vi "thermalCamera.vi"() -> ()   [LabVIEW 2025]
panel:
  out "Image":T1(plugin-control)
  out "IP address":string
  out "Output":string
  in  "Flag":bool
  in  "Stop recording":bool
  in  "Stop Preview":bool
  in  "Focus":dbl(slide) scale=0.0..100.0
  in  "Record":bool
  out "?":string
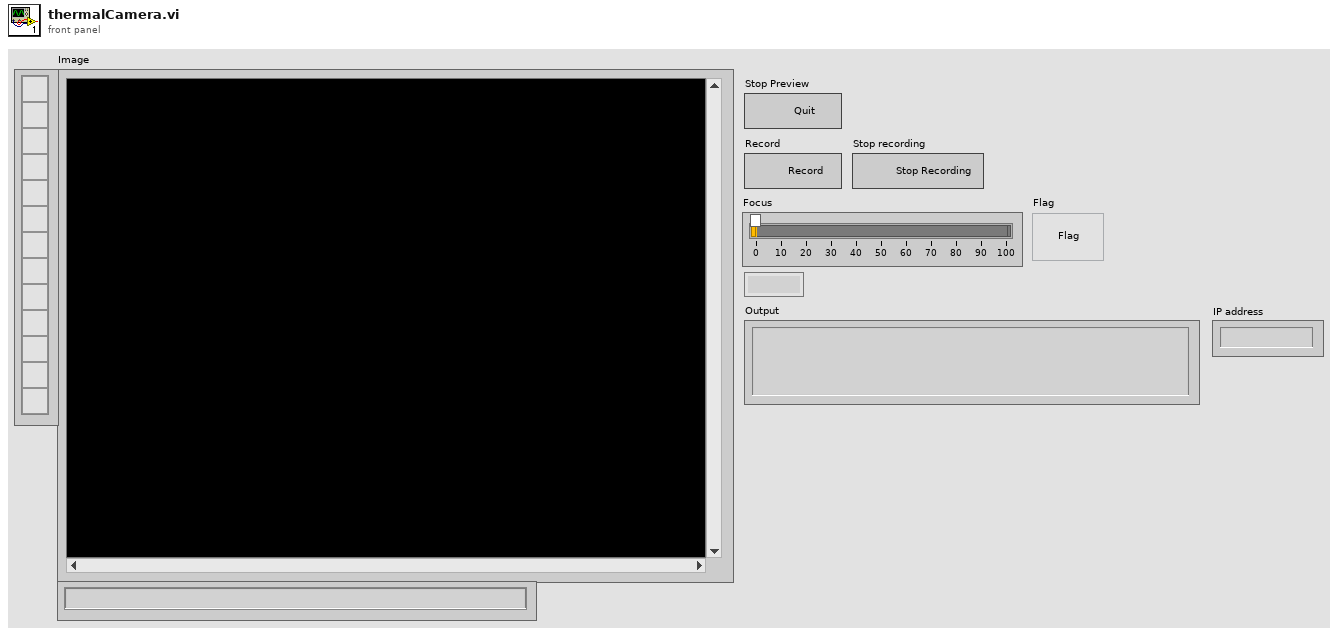
[diagram p1: front panel]
types:
  T1 = typedef "IMAQ Image.ctl" = refnum<image>
  T2 = enum16{"open", "replace", "create", "open or create", "replace or create", "replace or create with confirmation"}
  T3 = enum16{"big-endian, network order", "native, host order", "little-endian"}
  T4 = enum16{"Standard", "Buffered", "CRLF", "Immediate"}
  T5 = typedef "Image Type" = u32
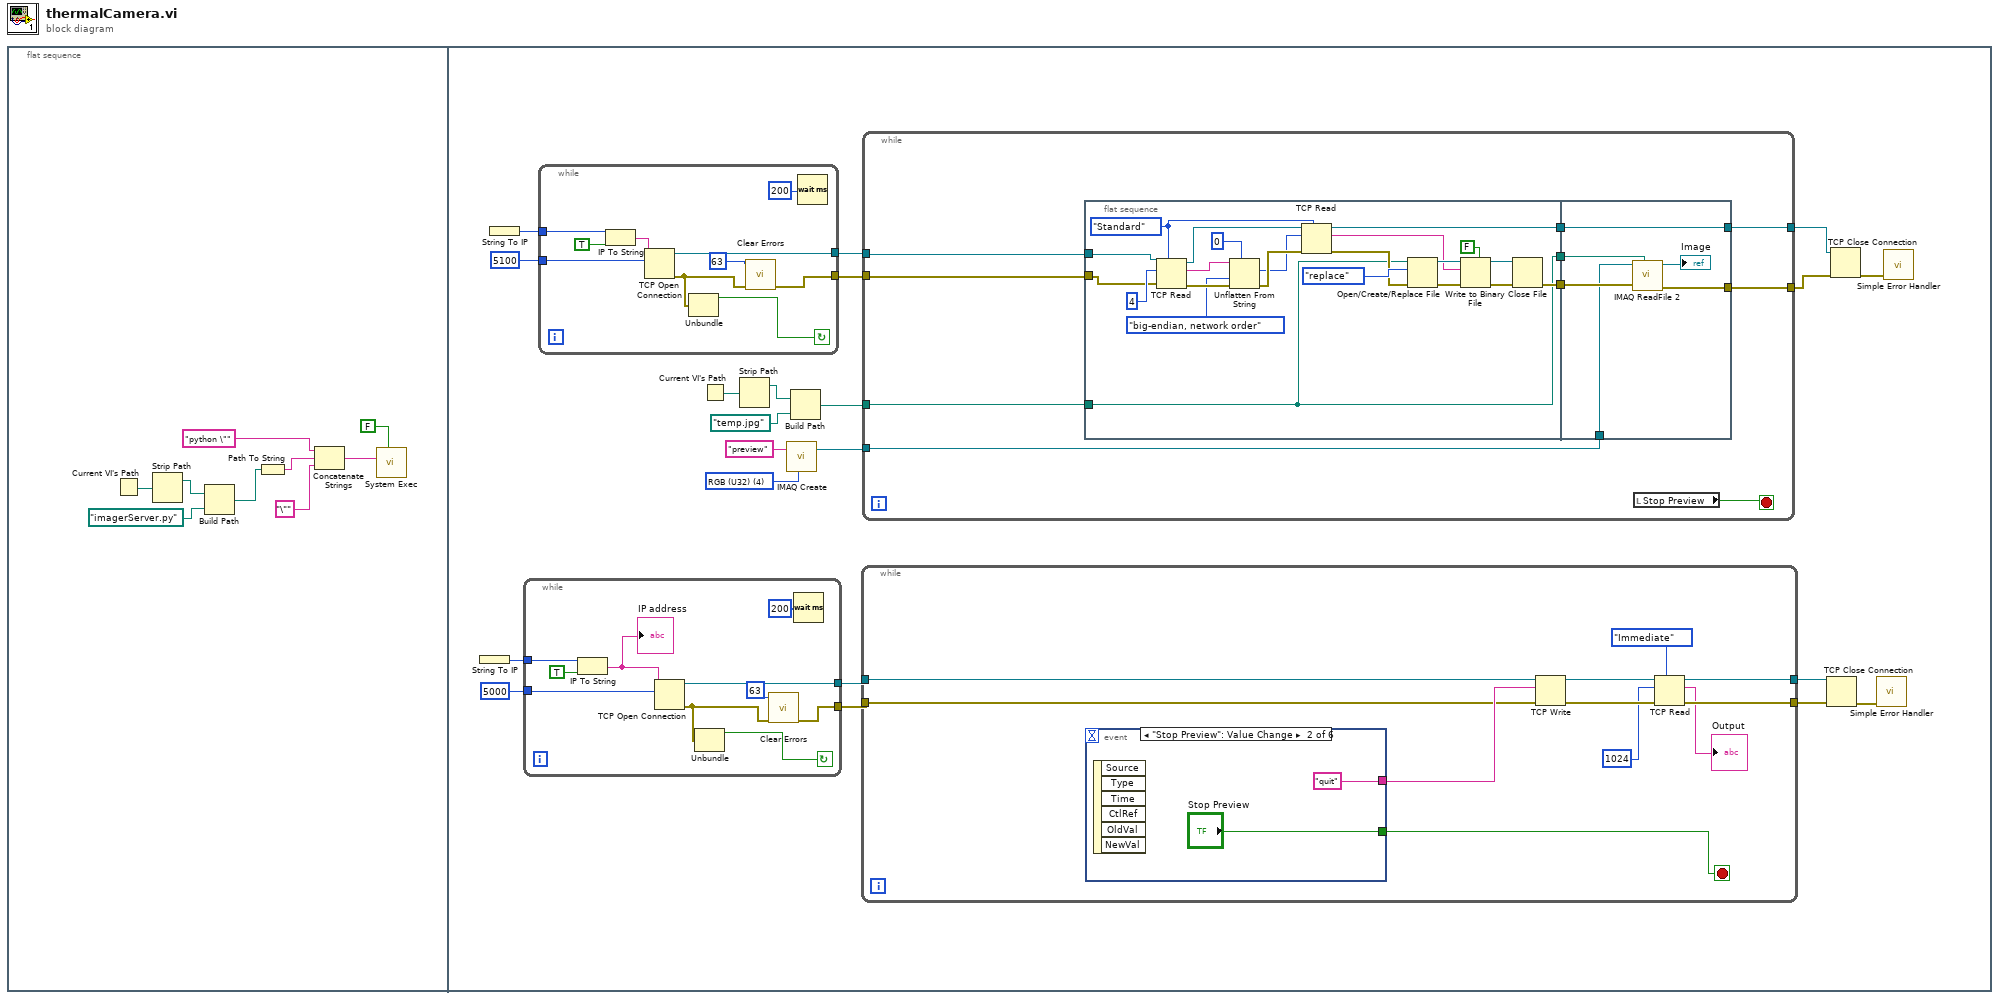
[diagram p0: block diagram]
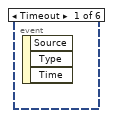
[diagram p2: hidden frame]
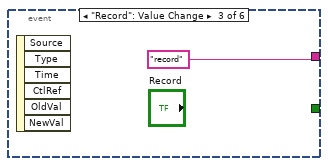
[diagram p3: hidden frame]
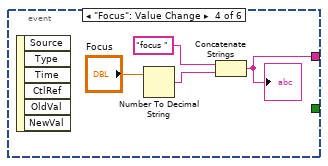
[diagram p4: hidden frame]
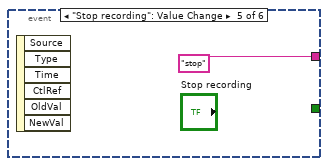
[diagram p5: hidden frame]
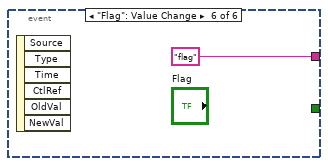
[diagram p6: hidden frame]
diagram:
  n1 = flat-sequence {
    frame #0 {
      n2 = Current VI's Path() -> (path=w4:path)
      n3 = Strip Path(path=w4) -> (stripped path=w5:path)  [unwired: 1 out]
      n4 = Build Path(base path=w5, name or relative path=path "imagerServer.py") -> (appended path=w2:path)
      n5 = Path To String(path=w2) -> (string=w8:string)
      n6 = Concatenate Strings("python \"" ("string"), w8, "\"" ("string")) -> (w7:string)
      n7 = call <vilib>:"System Exec.vi"("wait until completion? (T)"=FALSE, "command line"=w7) -> ()  [unwired: 6 in, 4 out]
    }
    frame #1 {
      w18 = T5 4 items=["Grayscale (U8)", "Grayscale (I16)", "Grayscale (SGL)", "Complex (CSG)", "RGB (U32)", "HSL (U32)", "RGB (U64)", "Grayscale (U16)"] ("Image Type")
      n8 = String To IP() -> (0:w15:u32)  [unwired: 1 in]
      n9 = String To IP() -> (0:w13:u32)  [unwired: 1 in]
      n10 = while {
        tunnel: [w44] -> w17
        tunnel: [w50] -> w16
        tunnel: w15 -> [w48]
        tunnel: u16 5000 ("remote port or service name") -> [w46]
        stop <- w41 continue-if-true
        n11 = IP To String(1:TRUE ("dot notation? (F)"), 2:w48) -> (0:w49:string)
        "IP address" <- w49
        n12 = TCP Open Connection(address=w49, remote port or service name=w46) -> (connection ID=w50:refnum<k5>, error out=w45:errorcluster)  [unwired: 3 in]
        n13 = Unbundle(w45) -> ("status"=w41:bool)  [unwired: 2 out]
        n14 = call <vilib>:"Clear Errors.vi"("error in (no error)"=w45, "specific error code to clear (0: all)"=63) -> ("error out"=w44:errorcluster)  [unwired: 4 in, 1 out]
        n15 = Wait (ms)(milliseconds to wait=u32 200) -> ()  [unwired: 1 out]
      }
      n16 = while {
        tunnel: w13 -> [w40]
        tunnel: [w34] -> w12
        tunnel: [w38] -> w11
        tunnel: u16 5100 ("remote port or service name") -> [w36]
        stop <- w31 continue-if-true
        n17 = IP To String(1:TRUE ("dot notation? (F)"), 2:w40) -> (0:w39:string)
        n18 = TCP Open Connection(address=w39, remote port or service name=w36) -> (connection ID=w38:refnum<k5>, error out=w35:errorcluster)  [unwired: 3 in]
        n19 = Unbundle(w35) -> ("status"=w31:bool)  [unwired: 2 out]
        n20 = call <vilib>:"Clear Errors.vi"("error in (no error)"=w35, "specific error code to clear (0: all)"=63) -> ("error out"=w34:errorcluster)  [unwired: 4 in, 1 out]
        n21 = Wait (ms)(milliseconds to wait=u32 200) -> ()  [unwired: 1 out]
      }
      n22 = Current VI's Path() -> (path=w29:path)
      n23 = Strip Path(path=w29) -> (stripped path=w30:path)  [unwired: 1 out]
      n24 = call "IMAQ Create"("Image Name"="preview", "Image Type"=w18) -> ("New Image"=w25:T1)  [unwired: 3 in, 1 out]
      n25 = Build Path(base path=w30, name or relative path=path "temp.jpg") -> (appended path=w28:path)
      n26 = while {
        tunnel: [w98] -> w21
        tunnel: [w96] -> w22
        tunnel: w17 -> [w94]
        tunnel: w16 -> [w93]
        stop <- w89 stop-if-true
        n27 = event shown="[1] \"Stop Preview\": Value Change" {
          selector: _ -> [_ _ _ _ _ _]
          dyn-events: _ -> [_ _ _ _ _ _]
          timeout: _ -> [_ _ _ _ _ _]
          tunnel: [_ "quit" "record" w104 "stop" "flag"] -> w95
          tunnel: [_ "Stop Preview" _ _ _ _] -> w89
          event Timeout {
            n28 = event-data() -> ()  [unwired: 1 in, 3 out]
          }
          event "Stop Preview": Value Change {
            n29 = event-data() -> ()  [unwired: 1 in, 6 out]
          }
          event "Record": Value Change {
            n30 = event-data() -> ()  [unwired: 1 in, 6 out]
          }
          event "Focus": Value Change {
            n31 = event-data() -> ()  [unwired: 1 in, 6 out]
            n32 = Number To Decimal String(number="Focus") -> (decimal integer string=w106:string)  [unwired: 1 in]
            n33 = Concatenate Strings("focus ", w106) -> (w104:string)
            "?" <- w104
          }
          event "Stop recording": Value Change {
            n34 = event-data() -> ()  [unwired: 1 in, 6 out]
          }
          event "Flag": Value Change {
            n35 = event-data() -> ()  [unwired: 1 in, 6 out]
          }
        }
        n36 = TCP Write(connection ID=w93, data in=w95, error in (no error)=w94) -> (connection ID out=w97:refnum<k5>, error out=w99:errorcluster)  [unwired: 1 in, 1 out]
        n37 = TCP Read(connection ID=w97, bytes to read=1024, error in (no error)=w99, 7:T4."Immediate" ("mode (standard)")) -> (connection ID out=w96:refnum<k5>, data out=→"Output":string, error out=w98:errorcluster)  [unwired: 1 in]
      }
      n38 = while {
        tunnel: w25 -> [w55]
        tunnel: [w56] -> w26
        tunnel: [w60] -> w27
        tunnel: w28 -> [w58]
        tunnel: w12 -> [w53]
        tunnel: w11 -> [w52]
        stop <- w51 stop-if-true
        n39 = flat-sequence {
          tunnel: w58 -> [w64]
          tunnel: [w66] -> w59
          tunnel: [w65] -> w57
          tunnel: [w64] -> w54
          tunnel: w53 -> [w62]
          tunnel: w52 -> [w61]
          tunnel: [w88] -> w60
          tunnel: w59 -> [w88]
          tunnel: w57 -> [w87]
          tunnel: [w86] -> w56
          tunnel: w55 -> [w85]
          tunnel: w54 -> [w84]
          frame #0 {
            w75 = T4."Standard" ("mode (standard)")
            n40 = TCP Read(connection ID=w61, bytes to read=4, error in (no error)=w62, 7:w75) -> (connection ID out=w78:refnum<k5>, data out=w63:string, error out=w81:errorcluster)  [unwired: 1 in]
            n41 = Unflatten From String(type=0, binary string=w63, byte order (0:big-endian, network order)=T3."big-endian, network order", error in (no error)=w81) -> (value=w76:i32, error out=w77:errorcluster)  [unwired: 1 in, 1 out]
            n42 = TCP Read(connection ID=w78, bytes to read=w76, error in (no error)=w77, 7:w75) -> (connection ID out=w66:refnum<k5>, data out=w71:string, error out=w73:errorcluster)  [unwired: 1 in]
            n43 = Open/Create/Replace File(file path (use dialog)=w64, error in=w73, operation (0:open)=T2."replace") -> (refnum out=w72:refnum<file>, error out=w69:errorcluster)  [unwired: 3 in, 1 out]
            n44 = Write to Binary File(file (use dialog)=w72, data=w71, error in=w69, 5:FALSE ("prepend array or string size? (T)")) -> (refnum out=w67:refnum<file>, error out=w68:errorcluster)  [unwired: 2 in, 1 out]
            n45 = Close File(refnum=w67, error in=w68) -> (error out=w65:errorcluster)  [unwired: 1 out]
          }
          frame #1 {
            n46 = call "IMAQ ReadFile 2"("File Path"=w84, "error in (no error)"=w87, "Image"=w85) -> ("error out"=w86:errorcluster, "Image Out"=→"Image":T1)  [unwired: 4 in, 3 out]
          }
        }
        n47 = local read "Stop Preview"() -> (w51:bool)
      }
      n48 = TCP Close Connection(connection ID=w22, error in (no error)=w21) -> (error out=w23:errorcluster)  [unwired: 1 in, 1 out]
      n49 = TCP Close Connection(connection ID=w27, error in (no error)=w26) -> (error out=w24:errorcluster)  [unwired: 1 in, 1 out]
      n50 = call <vilib>:"Simple Error Handler.vi"("error in (no error)"=w23) -> ()  [unwired: 4 in, 5 out]
      n51 = call <vilib>:"Simple Error Handler.vi"("error in (no error)"=w24) -> ()  [unwired: 4 in, 5 out]
    }
  }
